vi "logical_series.resolve_batch.vi"(7 "tags":map{string, string}(c390), 8 "error in":errorcluster, 9 "name":string, 10 "datasource":string, 11 "Nominal Client in":refnum<class "Nominal Client.lvclass">) -> (0 "error out":errorcluster, 2 "Response":string, 3 "Nominal Client out":refnum<class "Nominal Client.lvclass">)   [LabVIEW 2020, in "Nominal Client.lvclass"]
doc: "Resolves groups of channels, datasources and tags into logical series rids. An error response is provided if the channel + datasource + tag cannot be resolved into a logical series rid."
uses:
  Nominal Client.lvclass
  d51cee68-3910-4483-a6bc-435354615454.vi
  5272cbb0-1055-44a7-a196-32070c1239e9.vi
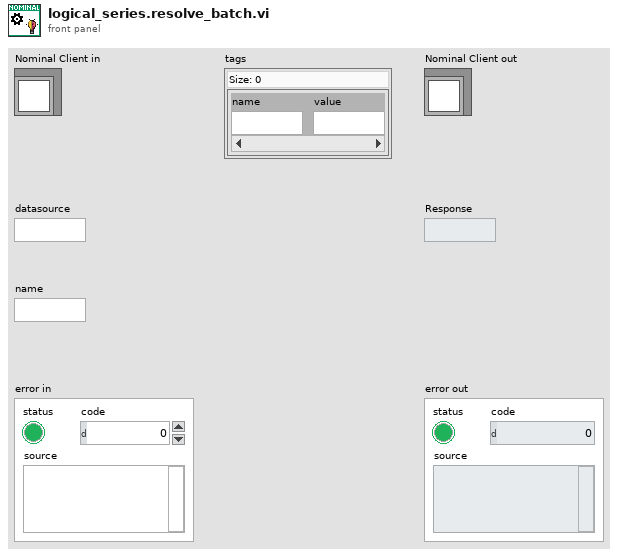
[diagram p1: front panel]
types:
  T1 = cluster{"name":string, "datasource":string, "tags":string}
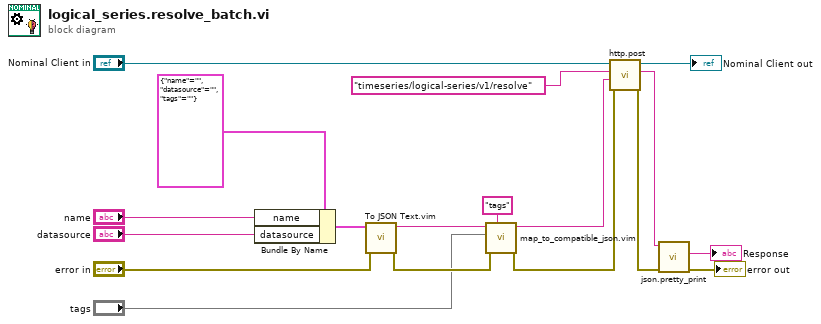
[diagram p0: block diagram]
diagram:
  n1 = Bundle By Name(cluster=T1 {"name"="", "datasource"="", "tags"=""}, "name"="name", "datasource"="datasource") -> (w5:T1)
  n2 = call "To JSON Text.vim"("error in (no error)"="error in", "Anything"=w5) -> ("error out"=w10:errorcluster, "<JSON>"=w13:string)  [unwired: 8 in]
  n3 = call "map_to_compatible_json.vim"("JSON Path"="tags", "error in"=w10, "Map"="tags", "JSON in"=w13) -> ("error out"=w11:errorcluster, "JSON out"=w12:string)  [unwired: 6 in]
  n4 = call "http.post.vi"("error in"=w11, "Request body"=w12, "Path"="timeseries/logical-series/v1/resolve", "Nominal Client in"="Nominal Client in") -> ("error out"=w2:errorcluster, "Response"=w4:string, "Nominal Client out"=→"Nominal Client out":refnum<class "Nominal Client.lvclass">)  [unwired: 4 in, 1 out]
  n5 = call "json.pretty_print.vi"("error in"=w2, "JSON in"=w4) -> ("error out"=→"error out":errorcluster, "Pretty JSON Out"=→"Response":string)  [unwired: 8 in]
